vi "set TXP Resolution BandWidth.vi"(8 "error in (no error)":errorcluster, 10 "BW Value (Hz)":dbl format="%#_6p", 11 "Interface_Spectrum in":refnum<class "Interface_Spectrum.lvclass">) -> (0 "error out":errorcluster, 3 "Interface_Spectrum out":refnum<class "Interface_Spectrum.lvclass">)   [LabVIEW 2023, in "Spectrum Analyzer.lvlib" / "Interface_Spectrum.lvclass"]
uses:
  Interface_Spectrum.lvclass
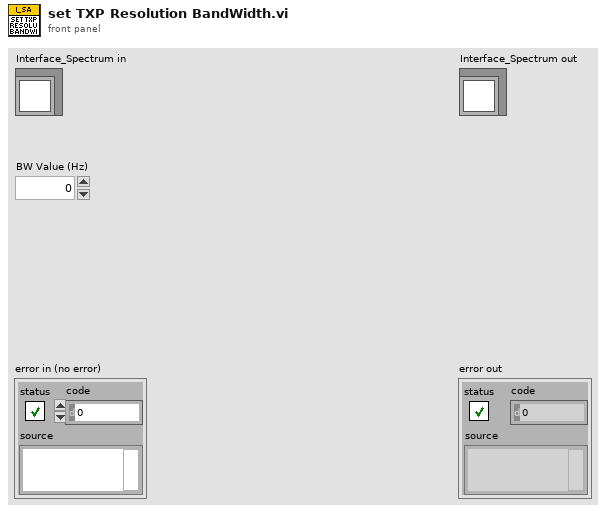
[diagram p1: front panel]
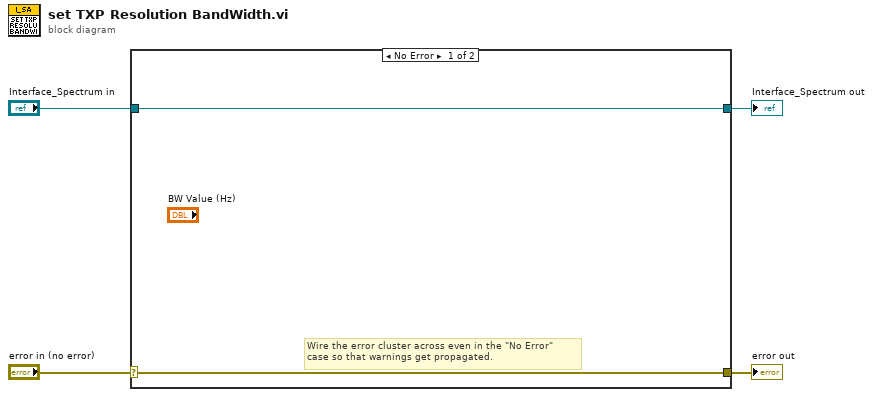
[diagram p0: block diagram]
diagram:
  n1 = case shown="No Error" "error in (no error)" {
    selector: "error in (no error)" -> [w5 w8]
    tunnel: [w5 w8] -> w3
    tunnel: [w6 w7] -> w1
    tunnel: "Interface_Spectrum in" -> [w6 w7]
    frame No Error {
      # "Wire the error cluster across even in the \"No Error\"\ncase so that warnings get propagated."
    }
    frame Error {
    }
  }
  "error out" <- w3
  "Interface_Spectrum out" <- w1
